vi "Lookup Target ID.vi"(8 "error in (no error)":errorcluster, 10 "Target Name":string, 11 "VolatusAPI in":refnum<class "VolatusAPI.lvclass">) -> (0 "error out":errorcluster, 1 "Type":T1=enum."Node", 2 "Target ID":u32, 3 "VolatusAPI out":refnum<class "VolatusAPI.lvclass">)   [LabVIEW 2020, in "Volatus.lvlib" / "VolatusAPI.lvclass"]
uses:
  VolatusAPI.lvclass
  VolatusConfig/Target Type.ctl
  VolatusAPI.lvclass/VolatusAPI.ctl
  VolatusConfig/VolatusConfig.lvlib
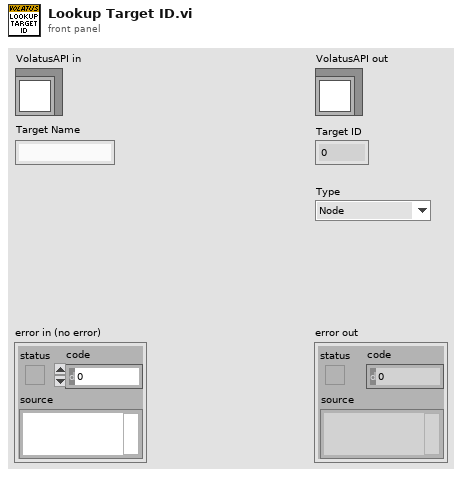
[diagram p1: front panel]
types:
  T1 = typedef "VolatusConfig.lvlib/Target Type.ctl" = enum16{"Unknown", "Node", "Group"}
  T2 = typedef "VolatusConfig.lvlib/Target Info.ctl" = cluster{"ID":u32, "Type":T1}
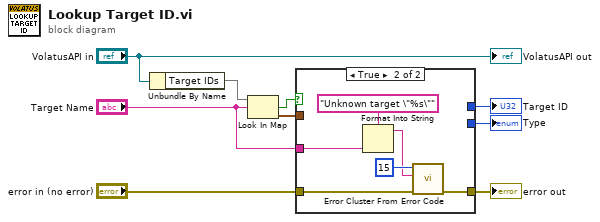
[diagram p0: block diagram]
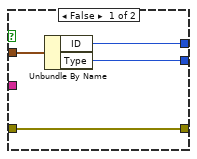
[diagram p2: hidden frame]
diagram:
  n1 = Unbundle By Name("VolatusAPI in") -> ("Target IDs"=w8:map{string, T2})
  n2 = Look In Map(map=w8, key="Target Name") -> (key not found?=w7:bool, value=w6:T2)  [unwired: 1 in]
  n3 = case shown="True" w7 {
    tunnel: w6 -> [w12 _]
    tunnel: "error in (no error)" -> [w13 w18]
    tunnel: [w13 w19] -> w4
    tunnel: [w11 _] -> w3
    tunnel: "Target Name" -> [_ w15]
    tunnel: [w10 _] -> w1
    frame False {
      n4 = Unbundle By Name(w12) -> ("ID"=w11:u32, "Type"=w10:T1)
    }
    frame True {
      n5 = Format Into String(format string="Unknown target \"%s\"", w15) -> (resulting string=w14:string)  [unwired: 2 in, 1 out]
      n6 = call <vilib>:"Error Cluster From Error Code.vi"("error in (no error)"=w18, "error message (\"\")"=w14, "error code (0)"=15) -> ("error out"=w19:errorcluster)  [unwired: 6 in]
    }
  }
  "error out" <- w4
  "Target ID" <- w3
  "Type" <- w1
  "VolatusAPI out" <- "VolatusAPI in"
